vi "Write Python Function Name.vi"(8 "error in":errorcluster, 10 "Python Function Name":string, 11 "Virtual Instrument in":refnum<class "Virtual Instrument.lvclass">) -> (0 "error out":errorcluster, 3 "Virtual Instrument out":refnum<class "Virtual Instrument.lvclass">)   [LabVIEW 2026, in "Virtual Instrument.lvclass"]
doc: "Data accessor."
uses:
  Virtual Instrument.lvclass
  Virtual Instrument.lvclass/Virtual Instrument.ctl
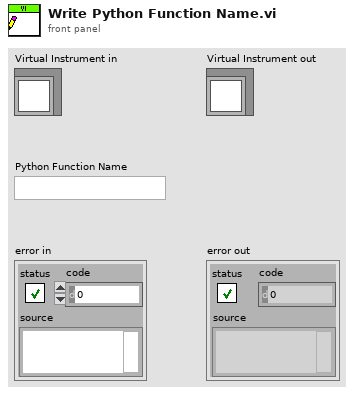
[diagram p1: front panel]
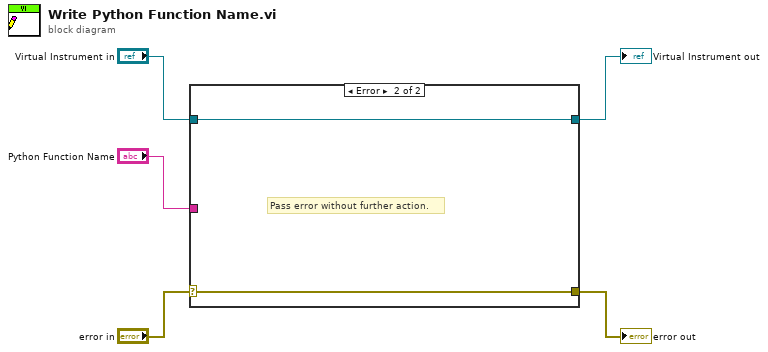
[diagram p0: block diagram]
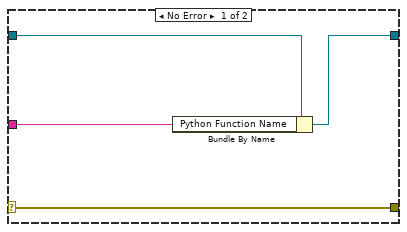
[diagram p2: hidden frame]
diagram:
  n1 = case shown="Error" "error in" {
    selector: "error in" -> [w9 w11]
    tunnel: [w9 w11] -> w4
    tunnel: [w7 w10] -> w2
    tunnel: "Virtual Instrument in" -> [w8 w10]
    tunnel: "Python Function Name" -> [w6 _]
    frame No Error {
      n2 = Bundle By Name(cluster=w8, "Python Function Name"=w6) -> (w7:refnum<class "Virtual Instrument.lvclass">)
    }
    frame Error {
      # "Pass error without further action."
    }
  }
  "error out" <- w4
  "Virtual Instrument out" <- w2
